vi "example test.vi"() -> ()   [LabVIEW 2013, in "TEC tests.lvlib"]
uses:
  TEC tests.lvlib
  configuration/TEC configuration.lvclass
  execution/TEC runtime.lvclass
  configuration/TEC configuration.lvclass/TEC configuration.ctl
  <vilib>/NI/Tag Bus/table/data polymorphs/write one/write Double.vi
  <vilib>/NI/Tag Bus/table/data polymorphs/write one/write Array of U64.vi
  <vilib>/NI/Tag Bus/table/data polymorphs/read one/read Array of U64.vi
  <vilib>/NI/Tag Bus/table/data polymorphs/read one/read Double.vi
  configuration/Write receive on port.vi
  configuration/Write send from port.vi
  configuration/Write send to address.vi
  configuration/Write send to port.vi
  <vilib>/NI/Tag Bus/table/data table.lvlib
  <vilib>/ptbypt/NI_PtbyPt.lvlib
  <vilib>/NI/Configuration Framework/serializable configuration/NISE_CEF_serializable configuration.lvclass
panel:
  out "value rx":u64[](array[numeric])
  in  "value":u64[](array[numeric])
  out "duration avg":dbl
  in  "millisecond multiple":u32=100
  out "duration":dbl
  out "timeout count":u16
  out "final":errorcluster
  out "value rx":dbl
  in  "value tx":dbl
  in  "stop":bool
  out "init err":errorcluster
  in  "ch count":i32=100
  out "serialization problem":errorcluster
  out "invalid configuration":errorcluster
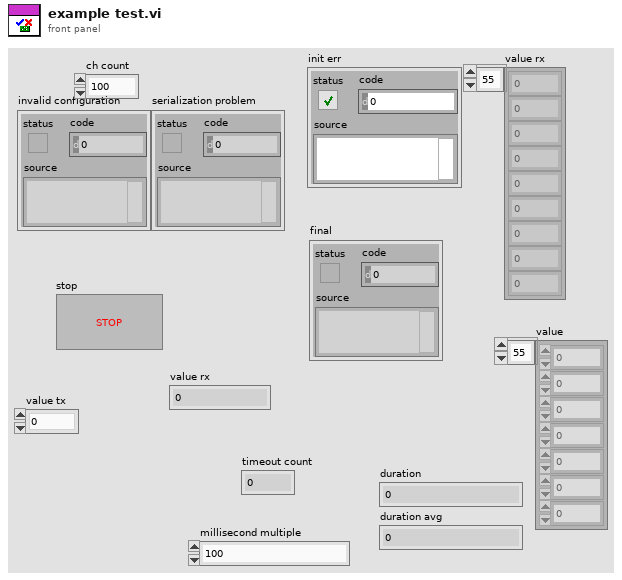
[diagram p1: front panel]
types:
  T1 = typedef "TBM channel.lvclass/data tables.ctl" = cluster{"input data":T2, "processing parameter":T2, "processing result":T2, "output data":T2}
  T2 = typedef "tag bus.lvlib/dictionary table pair.ctl" = cluster{"data dictionary":refnum<class "data dictionary.lvclass">, "data table":T3}
  T3 = typedef "tag bus.lvlib/data table.lvlib/data table.ctl" = cluster{"Double":dbl[], "Single":sgl[], "I64":i64[], "I32":i32[], "I16":i16[], "I8":i8[], "U64":u64[], "U32":u32[], "U16":u16[], "U8":u8[], "Boolean":bool[], "String":string[], "Array of Double":cluster{"DBL Array":dbl[]}[], "Array of Single":cluster{"SGL Array":sgl[]}[], "Array of I64":cluster{"I64 Array":i64[]}[], "Array of I32":cluster{"I32 Array":i32[]}[], "Array of I16":cluster{"I16 Array":i16[]}[], "Array of I8":cluster{"I8 Array":i8[]}[], "Array of U64":cluster{"U64 Array":u64[]}[], "Array of U32":cluster{"U32 Array":u32[]}[], "Array of U16":cluster{"U16 Array":u16[]}[], "Array of U8":cluster{"U8 Array":u8[]}[], "Array of Boolean":cluster{"Boolean Array":bool[]}[], "Array of String":cluster{"String Array":string[]}[]}
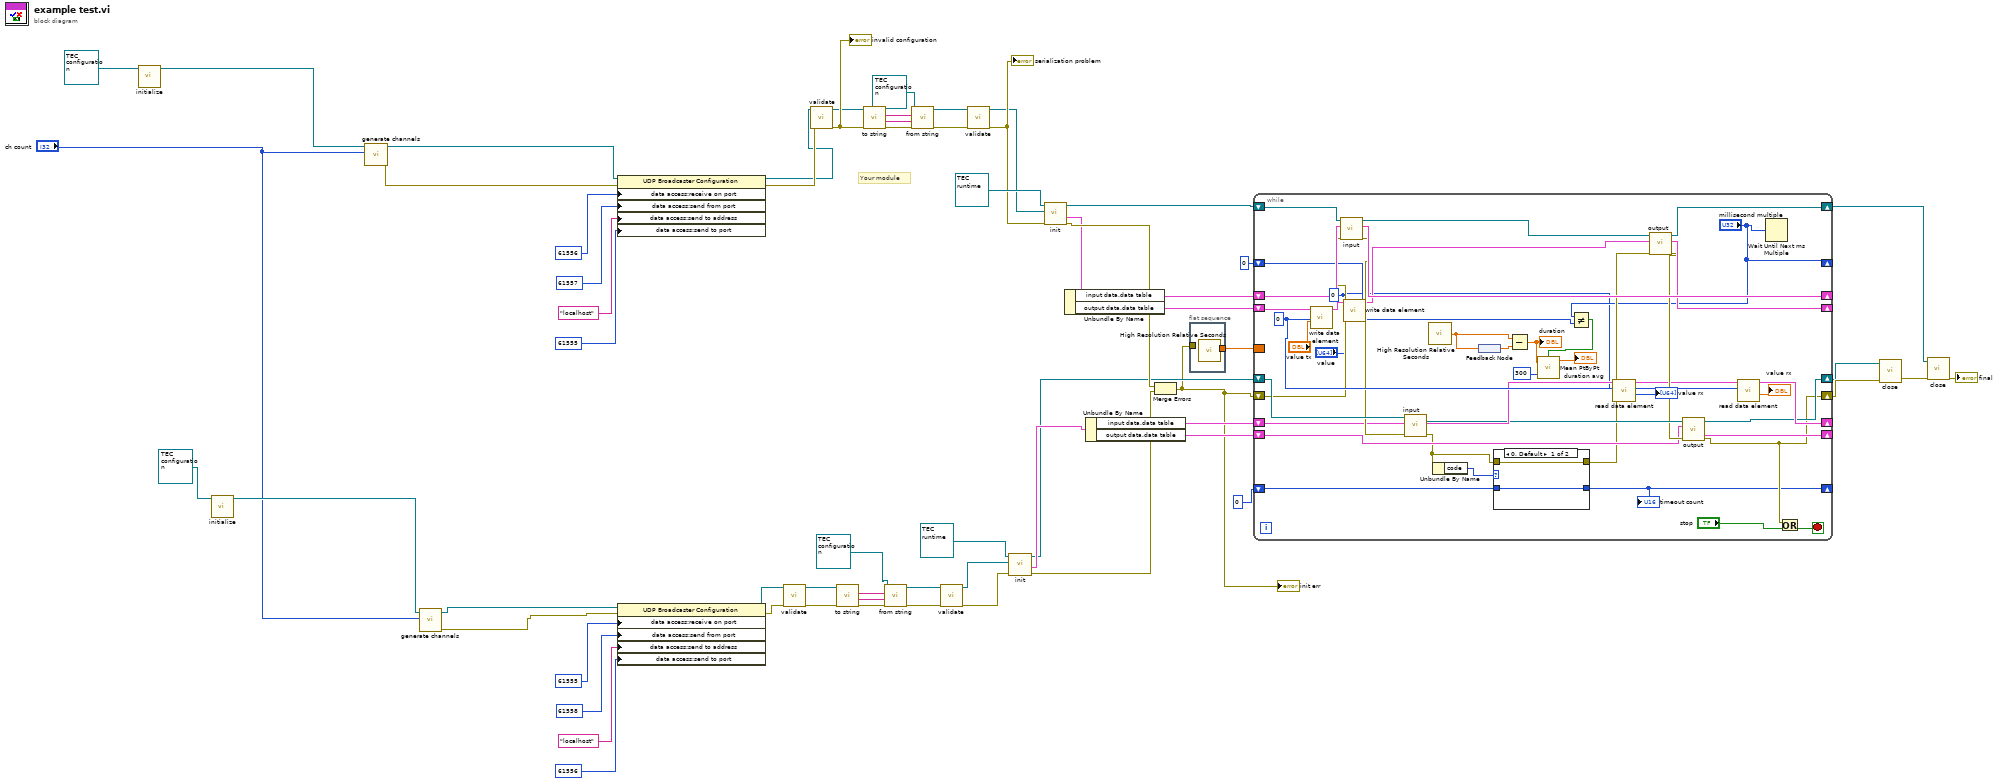
[diagram p0: block diagram]
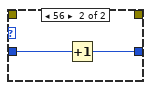
[diagram p2: hidden frame]
diagram:
  # "Your module"
  n1 = call <vilib>:"initialize.vi"("configuration in"=refnum<class "TEC configuration.lvclass"> refnum ("tag bus configurable plugin module configuration")) -> ("configuration out"=w8:refnum<class "TEC configuration.lvclass">)  [unwired: 8 in, 2 out]
  n2 = call <vilib>:"initialize.vi"("configuration in"=refnum<class "TEC configuration.lvclass"> refnum ("tag bus configurable plugin module configuration")) -> ("configuration out"=w4:refnum<class "TEC configuration.lvclass">)  [unwired: 8 in, 2 out]
  n3 = call "generate channels.vi"("ch count"="ch count", "TEC configuration in"=w8) -> ("error out"=w52:errorcluster, "TEC configuration out"=w50:refnum<class "TEC configuration.lvclass">)  [unwired: 8 in]
  n4 = call "generate channels.vi"("ch count"="ch count", "TEC configuration in"=w4) -> ("error out"=w6:errorcluster, "TEC configuration out"=w5:refnum<class "TEC configuration.lvclass">)  [unwired: 8 in]
  n5 = property class="UDP Broadcaster Configuration"(reference=w50, error in=w52, "data access:receive on port"=u16 61556 ("send from port"), "data access:send from port"=u16 61557 ("send to port"), "data access:send to address"="localhost" ("send to address"), "data access:send to port"=u16 61555 ("receive on port")) -> (reference out=w49:refnum<class "TEC configuration.lvclass">, error out=w51:errorcluster)
  n6 = property class="UDP Broadcaster Configuration"(reference=w5, error in=w6, "data access:receive on port"=u16 61555 ("send from port"), "data access:send from port"=u16 61558 ("send to port"), "data access:send to address"="localhost" ("send to address"), "data access:send to port"=u16 61556 ("receive on port")) -> (reference out=w30:refnum<class "TEC configuration.lvclass">, error out=w31:errorcluster)
  n7 = call-dynamic "validate.vi"("error in"=w31, "TEC configuration in"=w30) -> ("error out"=w32:errorcluster, "TEC configuration out"=w38:refnum<class "TEC configuration.lvclass">)  [unwired: 8 in]
  n8 = call-dynamic "validate.vi"("error in"=w51, "TEC configuration in"=w49) -> ("error out"=w62:errorcluster, "TEC configuration out"=w40:refnum<class "TEC configuration.lvclass">)  [unwired: 8 in]
  "invalid configuration" <- w62
  n9 = call-dynamic "to string.vi"("error in"=w32, "TEC configuration in"=w38) -> ("error out"=w35:errorcluster, "data"=w34:string, "version"=w33:string)  [unwired: 6 in, 1 out]
  n10 = call-dynamic "to string.vi"("error in"=w62, "TEC configuration in"=w40) -> ("error out"=w59:errorcluster, "data"=w60:string, "version"=w61:string)  [unwired: 6 in, 1 out]
  n11 = call-dynamic "from string.vi"("error in"=w35, "data"=w34, "version"=w33, "TEC configuration in"=refnum<class "TEC configuration.lvclass"> refnum) -> ("error out"=w37:errorcluster, "TEC configuration out"=w36:refnum<class "TEC configuration.lvclass">)  [unwired: 6 in]
  n12 = call-dynamic "from string.vi"("error in"=w59, "data"=w60, "version"=w61, "TEC configuration in"=refnum<class "TEC configuration.lvclass"> refnum) -> ("error out"=w57:errorcluster, "TEC configuration out"=w58:refnum<class "TEC configuration.lvclass">)  [unwired: 6 in]
  n13 = call-dynamic "validate.vi"("error in"=w37, "TEC configuration in"=w36) -> ("error out"=w28:errorcluster, "TEC configuration out"=w27:refnum<class "TEC configuration.lvclass">)  [unwired: 8 in]
  n14 = call-dynamic "validate.vi"("error in"=w57, "TEC configuration in"=w58) -> ("error out"=w55:errorcluster, "TEC configuration out"=w54:refnum<class "TEC configuration.lvclass">)  [unwired: 8 in]
  "serialization problem" <- w55
  n15 = call-dynamic "init.vi"("error in"=w28, "TBM module configuration in"=w27, "TEC runtime in"=refnum<class "TEC runtime.lvclass"> refnum ("tag bus configurable plugin module")) -> ("error out"=w25:errorcluster, "data allocations"=w22:T1, "TEC runtime out"=w16:refnum<class "TEC runtime.lvclass">)  [unwired: 5 in, 1 out]
  n16 = call-dynamic "init.vi"("error in"=w55, "TBM module configuration in"=w54, "TEC runtime in"=refnum<class "TEC runtime.lvclass"> refnum ("tag bus configurable plugin module")) -> ("error out"=w26:errorcluster, "data allocations"=w23:T1, "TEC runtime out"=w17:refnum<class "TEC runtime.lvclass">)  [unwired: 5 in, 1 out]
  n17 = Unbundle By Name(w23) -> ("input data.data table"=w19:T3, "output data.data table"=w18:T3)
  n18 = Unbundle By Name(w22) -> ("input data.data table"=w21:T3, "output data.data table"=w20:T3)
  n19 = Merge Errors(w26, w25) -> (w1:errorcluster)
  "init err" <- w1
  n20 = flat-sequence {
    tunnel: [w63] -> w2
    tunnel: w1 -> [_]
    frame #0 {
      n21 = call <vilib>:"High Resolution Relative Seconds.vi"() -> ("relative seconds"=w63:dbl)
    }
  }
  n22 = while {
    shift-right: [w102] -> _
    shift-left: w21 -> [w93]
    shift-right: [w85] -> _
    shift-left: w20 -> [w82]
    shift-right: [w88] -> _
    shift-left: w18 -> [w104]
    shift-right: [w97] -> _
    shift-left: w19 -> [w98]
    shift-right: [w90] -> w12
    shift-left: w17 -> [w99]
    shift-right: [w86] -> w11
    shift-left: w16 -> [w96]
    shift-right: [w83] -> w15
    shift-left: w1 -> [w95]
    shift-right: [w78] -> _
    shift-left: u16 0 ("Numeric") -> [w77]
    shift-right: ["millisecond multiple"] -> _
    shift-left: u32 0 ("millisecond multiple") -> [w71]
    border: w2 -> [_]
    stop <- w105 stop-if-true
    w65 = 0 ("index")
    w100 = 0 ("index")
    n23 = call-poly <vilib>:"write data element.vi"("value"="value tx", "index"=w100, "data table in"=w104) -> ("data table out"=w89:T3)  [unwired: 8 in]
    n24 = call-dynamic "input.vi"("error in"=w95, "data table in"=w98, "TEC runtime in"=w99) -> ("error out"=w94:errorcluster, "data table out"=w97:T3, "TEC runtime out"=w91:refnum<class "TEC runtime.lvclass">)  [unwired: 6 in]
    n25 = call-poly <vilib>:"write data element.vi"("value"="value", "index"=w65, "data table in"=w89) -> ("data table out"=w68:T3)  [unwired: 8 in]
    n26 = call-dynamic "input.vi"("error in"=w94, "data table in"=w93, "TEC runtime in"=w96) -> ("error out"=w80:errorcluster, "data table out"=w92:T3, "TEC runtime out"=w87:refnum<class "TEC runtime.lvclass">)  [unwired: 6 in]
    n27 = call <vilib>:"High Resolution Relative Seconds.vi"() -> ("relative seconds"=w75:dbl)
    n28 = Unbundle By Name(w80) -> ("code"=w81:i32)
    n29 = feedback-in #1(w75) -> ()
    n30 = feedback #1() -> (w76:dbl)
    n31 = case shown="0, Default" w81 {
      tunnel: w80 -> [w108 _]
      tunnel: [w108 _] -> w79
      tunnel: [w107 w110] -> w78
      tunnel: w77 -> [w107 w109]
      frame 0, Default {
      }
      frame 56 {
        n32 = Increment(x=w109) -> (x+1=w110:u16)
      }
    }
    "timeout count" <- w78
    n33 = Subtract(x=w75, y=w76) -> (x-y=w74:dbl)
    "duration" <- w74
    n34 = Not Equal?(x="millisecond multiple", y=w71) -> (x != y?=w70:bool)
    n35 = call <vilib>:"Mean PtByPt.vi"("x"=w74, "sample length"=300, "initialize"=w70) -> ("mean"=→"duration avg":dbl)  [unwired: 1 in, 1 out]
    n36 = call-poly <vilib>:"read data element.vi"("index"=w65, "data table in"=w92) -> ("value"=→"value rx":u64[], "data table out"=w66:T3)  [unwired: 8 in]
    n37 = call-dynamic "output.vi"("error in"=w79, "data table in"=w68, "TEC runtime in"=w91) -> ("error out"=w84:errorcluster, "data table out"=w88:T3, "TEC runtime out"=w90:refnum<class "TEC runtime.lvclass">)  [unwired: 6 in]
    n38 = call-dynamic "output.vi"("error in"=w84, "data table in"=w82, "TEC runtime in"=w87) -> ("error out"=w83:errorcluster, "data table out"=w85:T3, "TEC runtime out"=w86:refnum<class "TEC runtime.lvclass">)  [unwired: 6 in]
    n39 = call-poly <vilib>:"read data element.vi"("index"=w100, "data table in"=w66) -> ("value"=→"value rx":dbl, "data table out"=w102:T3)  [unwired: 8 in]
    n40 = Wait Until Next ms Multiple(millisecond multiple="millisecond multiple") -> ()  [unwired: 1 out]
    n41 = Or(x=w83, y="stop") -> (x .or. y?=w105:bool)
  }
  n42 = call-dynamic "close.vi"("error in"=w15, "TEC runtime in"=w11) -> ("error out"=w14:errorcluster)  [unwired: 9 in]
  n43 = call-dynamic "close.vi"("error in"=w14, "TEC runtime in"=w12) -> ("error out"=→"final":errorcluster)  [unwired: 9 in]
